vi "Func - VarMan VI Error Cluster to Func Result Value.vi"(8 "VarMan VI error in":errorcluster) -> (0 "CE Function Result Value":i32)   [LabVIEW 2021]
doc: "This VI converts an error returned by a VarMan VI to the value returned by a FuncVI function. Refer to the VI help for more details.\n\n::: CalcExpress Toolkit :::\nCopyright (c) 2000-2026 Konstantin Shifershteyn. All rights reserved."
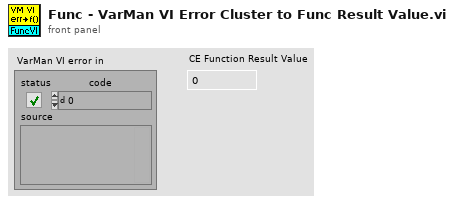
[diagram p1: front panel]
types:
  T1 = typedef "VarMan Error Code.ctl" = u16
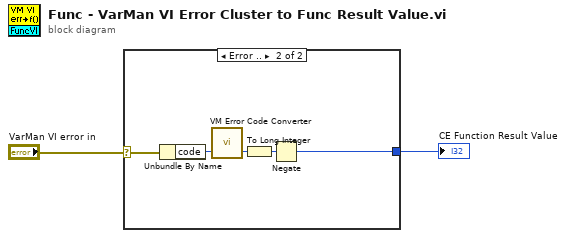
[diagram p0: block diagram]
diagram:
  n1 = case shown="Error .." "VarMan VI error in" {
    selector: "VarMan VI error in" -> [_ w4]
    tunnel: [_ w3] -> w1
    frame No Error {
    }
    frame Error {
      n2 = Unbundle By Name(w4) -> ("code"=w7:i32)
      n3 = call "VM Error Code Converter.vi"("VM VI error code in"=w7) -> ("VM Engine error code out"=w5:T1)  [unwired: 1 in, 1 out]
      n4 = To Long Integer(number=w5) -> (32bit integer=w6:i32)
      n5 = Negate(x=w6) -> (-x=w3:i32)
    }
  }
  "CE Function Result Value" <- w1
